vi "Test_pgADONet.vi"() -> ()   [LabVIEW 2026]
uses:
  <vilib>/Viviota/shared/ORM.lvlibp/TypeMap/TypeMap.lvclass
  <vilib>/Viviota/shared/ORM_ADONetCore.lvlibp/ADOMapper/ADOMapper.lvclass
  C:/Program Files/National Instruments/LabVIEW 2026/vi.lib/Viviota/shared/ORM.lvlibp/SqlMapper/SqlMapper.lvclass
  dotNetCore/ORM_DBC_Npgsql_netCore/DBC.lvclass
  C:/Program Files/National Instruments/LabVIEW 2026/vi.lib/Viviota/shared/ORM.lvlibp/DbConnection/DbConnection.lvclass
  <vilib>/Viviota/shared/ORM_lib.lvlibp/ObjectRow/ObjectLUT.lvclass
  <vilib>/numeric/Random Number (Range) I64.vi
  <vilib>/numeric/Random Number (Range) DBL.vi
  f3693442-7653-4e44-a421-498bef5f0c13.vi
  <vilib>/Analysis/baseanly.llb/Mean (DBL).vi
  <vilib>/numeric/sub_Random U32.vi
  <vilib>/JDP Science/JSONtext/Variant to JSON Text.vi
  <vilib>/Viviota/shared/ORM_lib.lvlibp/ObjectRow/Write LUT.vi
  <vilib>/Viviota/shared/ORM.lvlibp/DbConnection/Write SupportTX.vi
  <vilib>/Viviota/shared/ORM.lvlibp/SqlMapper/Write DbConnection.vi
  <vilib>/Viviota/shared/ORM.lvlibp/TypeMap/Write Table Name.vi
  <vilib>/Viviota/shared/ORM.lvlibp/TypeMap/Write Autokey.vi
  <vilib>/Viviota/shared/ORM_lib.lvlibp/ObjectRow/Read LUT.vi
  <vilib>/JDP Science/JSONtext/LVClass Serializer/JSONtext LVClass Serializer.lvclass
  <vilib>/Analysis/NI_AALBase.lvlib
panel:
  out "Numeric 2":i32
  out "Numeric":i32
  out "mean 3":dbl format="%0.6f"
  out "mean 2":dbl format="%0.6f"
  out "mean":dbl format="%0.6f"
  out "x-y":dbl[](array[numeric])
  out "Array 2":dbl[](array[numeric])
  out "Array":dbl[](array[numeric])
  out "LUT 2":variant[](array[variant])
  out "LUT":variant[](array[variant])
  out "id":i32[](array[numeric])
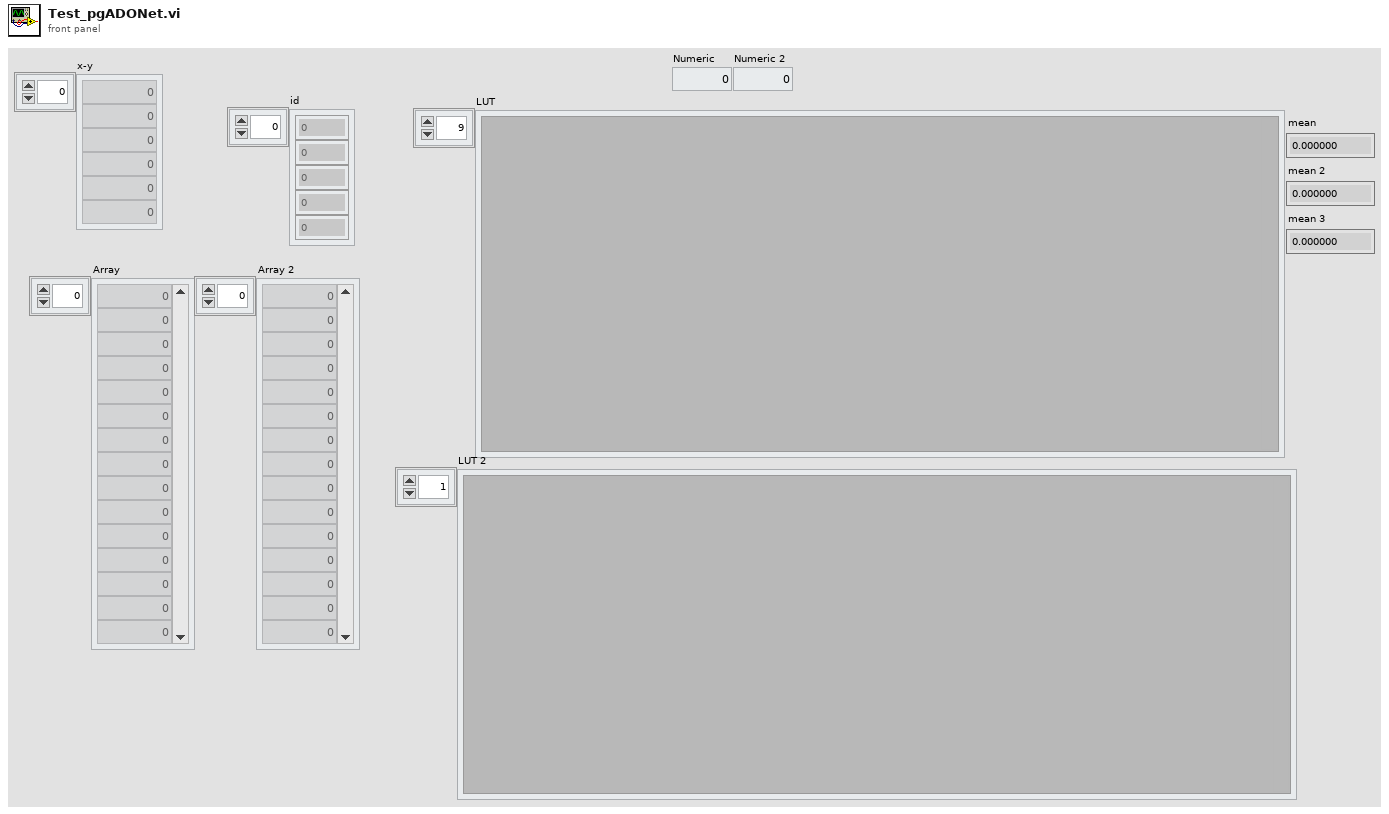
[diagram p1: front panel]
types:
  T1 = cluster{"Text":string, "Integer":i32, "dbl":dbl, "timestamp":timestamp}
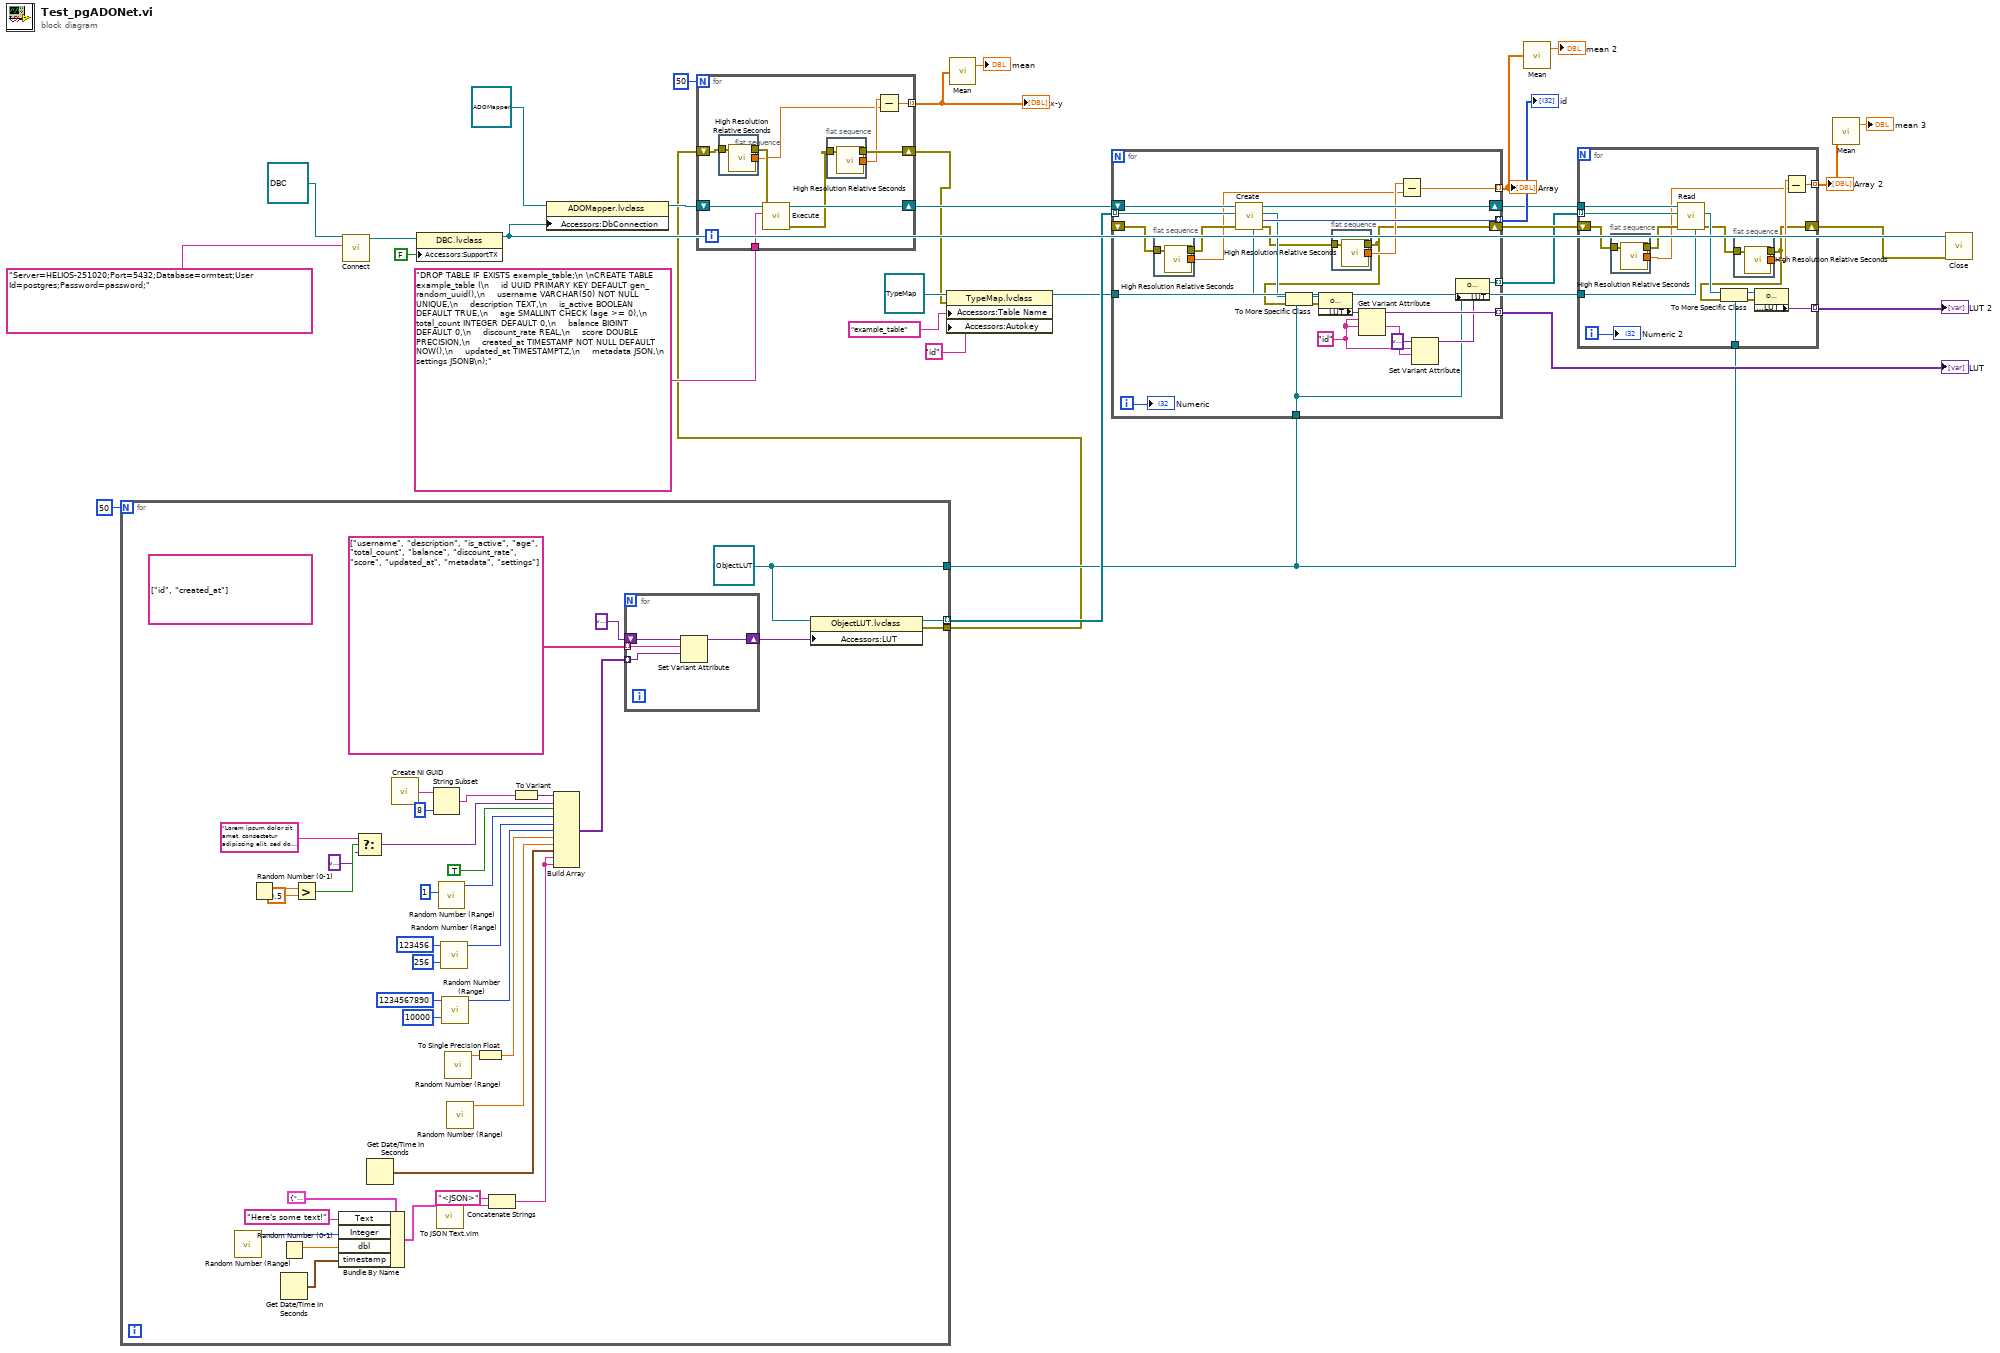
[diagram p0: block diagram]
diagram:
  n1 = for {
    N: 50 -> [_]
    tunnel: [w39] -> w26 mode=indexing
    tunnel: [w38] -> w16
    tunnel: [w33] -> w11
    w38 = refnum<class "ObjectLUT.lvclass"> refnum ("ORM_lib.lvlibp:ObjectLUT.lvclass")
    (unwired) string[] ["id", "created_at"]
    n2 = call-poly <vilib>:"Random Number (Range).vi"() -> ("number"=w46:i64)  [unwired: 11 in]
    n3 = Random Number (0-1)() -> (number: 0 to 1=w55:dbl)
    n4 = Random Number (0-1)() -> (number: 0 to 1=w47:dbl)
    n5 = Get Date/Time In Seconds() -> (seconds since 1Jan1904=w48:timestamp)
    n6 = Greater?(x=w55, y=0.5) -> (0:w53:bool)
    n7 = Bundle By Name(cluster=T1 {"Text"="This is a test", "Integer"=0, "dbl"=0.0, "timestamp"=timestamp(0 s since 1904-01-01)}, "Text"="Here's some text!", "Integer"=w46, "dbl"=w47, "timestamp"=w48) -> (w44:T1)
    n8 = Select(t="Lorem ipsum dolor sit amet, consectetur adipiscing elit, sed do eiusmod tempor incididunt ut labore et dolore magna aliqua", s=w53, f=variant) -> (s? t:f=w51:variant)
    n9 = Get Date/Time In Seconds() -> (seconds since 1Jan1904=w45:timestamp)
    n10 = call <vilib>:"Create NI GUID.vi"() -> ("NI GUID"=w71:string)
    n11 = String Subset(string=w71, length (rest)=8 ("length (rest)")) -> (substring=w66:string)  [unwired: 1 in]
    n12 = call "To JSON Text.vim"("Anything"=w44) -> ("<JSON>"=w37:string)  [unwired: 9 in, 1 out]
    n13 = call-poly <vilib>:"Random Number (Range).vi"("lower bound (-100)"=i64 1) -> ("number"=w63:i64)  [unwired: 10 in]
    n14 = call-poly <vilib>:"Random Number (Range).vi"("lower bound (-100)"=i64 256, "upper bound (100)"=i64 123456) -> ("number"=w62:i64)  [unwired: 9 in]
    n15 = call-poly <vilib>:"Random Number (Range).vi"("lower bound (-100)"=i64 10000, "upper bound (100)"=i64 1234567890) -> ("number"=w61:i64)  [unwired: 9 in]
    n16 = call-poly <vilib>:"Random Number (Range).vi"() -> ("number"=w59:dbl)  [unwired: 11 in]
    n17 = call-poly <vilib>:"Random Number (Range).vi"() -> ("number"=w57:dbl)  [unwired: 11 in]
    n18 = To Single Precision Float(number=w59) -> (single precision float=w58:sgl)
    n19 = Concatenate Strings("<JSON>" ("string"), w37) -> (w36:string)
    n20 = To Variant(anything=w66) -> (Variant=w65:variant)
    n21 = Build Array(w65, w51, TRUE, w63, w62, w61, w58, w57, w45, w36, w36) -> (w42:variant[])
    n22 = for {
      tunnel: string[] ["username", "description", "is_active", "age", "total_count", "balance", "discount_rate", "score", "updated_at", "metadata", "settings"] -> [w75] mode=indexing
      tunnel: w42 -> [w74] mode=indexing
      shift-right: [w73] -> w40
      shift-left: variant -> [w72]
      n23 = Set Variant Attribute(Variant=w72, name=w75, value=w74) -> (Variant out=w73:variant)  [unwired: 1 in, 2 out]
    }
    n24 = property class="ObjectLUT.lvclass"(reference=w38, "Accessors:LUT"=w40) -> (reference out=w39:refnum<class "ObjectLUT.lvclass">, error out=w33:errorcluster)  [unwired: 1 in]
  }
  n25 = call-dynamic "Connect.vi"("Connection String"="Server=HELIOS-251020;Port=5432;Database=ormtest;User Id=postgres;Password=password;", "PostgresqlConnection in"=refnum<class "DBC.lvclass"> refnum ("ORM_DBC_Npgsql_netCore.lvlib:DBC.lvclass")) -> ("PostgresqlConnection out"=w31:refnum<class "DBC.lvclass">)  [unwired: 8 in, 1 out]
  n26 = property class="DBC.lvclass"(reference=w31, "Accessors:SupportTX"=FALSE ("SupportTX")) -> (reference out=w27:refnum<class "DBC.lvclass">)  [unwired: 1 in, 1 out]
  n27 = property class="ADOMapper.lvclass"(reference=refnum<class "ADOMapper.lvclass"> refnum ("ORM_ADONetCore.lvlibp:ADOMapper.lvclass"), "Accessors:DbConnection"=w27) -> (reference out=w29:refnum<class "ADOMapper.lvclass">)  [unwired: 1 in, 1 out]
  n28 = for {
    N: 50 -> [_]
    tunnel: "DROP TABLE IF EXISTS example_table;\n \nCREATE TABLE example_table (\n    id UUID PRIMARY KEY DEFAULT gen_random_uuid(),\n    username VARCHAR(50) NOT NULL UNIQUE,\n    description TEXT,\n    is_active BOOLEAN DEFAULT TRUE,\n    age SMALLINT CHECK (age >= 0),\n    total_count INTEGER DEFAULT 0,\n    balance BIGINT DEFAULT 0,\n    discount_rate REAL,\n    score DOUBLE PRECISION,\n    created_at TIMESTAMP NOT NULL DEFAULT NOW(),\n    updated_at TIMESTAMPTZ,\n    metadata JSON,\n    settings JSONB\n);" ("sql") -> [w84]
    tunnel: [w76] -> w7 mode=indexing
    shift-right: [w83] -> w18
    shift-left: w29 -> [w85]
    shift-right: [w79] -> w10
    shift-left: w11 -> [w82]
    n29 = flat-sequence {
      tunnel: [w89] -> w77
      tunnel: w82 -> [w88]
      tunnel: [w88] -> w81
      frame #0 {
        n30 = call <vilib>:"High Resolution Relative Seconds.vi"() -> ("relative seconds"=w89:dbl)
      }
    }
    n31 = call-dynamic "Execute.vi"("error in (no error)"=w81, "sql"=w84, "ADOMapper in"=w85) -> ("error out"=w80:errorcluster, "ADOMapper out"=w83:refnum<class "ADOMapper.lvclass">)  [unwired: 6 in, 1 out]
    n32 = flat-sequence {
      tunnel: [w87] -> w78
      tunnel: w80 -> [w86]
      tunnel: [w86] -> w79
      frame #0 {
        n33 = call <vilib>:"High Resolution Relative Seconds.vi"() -> ("relative seconds"=w87:dbl)
      }
    }
    n34 = Subtract(x=w78, y=w77) -> (x-y=w76:dbl)
  }
  "x-y" <- w7
  n35 = property class="TypeMap.lvclass"(reference=refnum<class "TypeMap.lvclass"> refnum ("TypeMap in"), error in=w10, "Accessors:Table Name"="example_table" ("Table Name"), "Accessors:Autokey"="id" ("Autokey")) -> (reference out=w17:refnum<class "TypeMap.lvclass">)  [unwired: 1 out]
  n36 = call-poly <vilib>:"Mean.vi"("X"=w7) -> ("mean"=→"mean":dbl)  [unwired: 1 out]
  n37 = for {
    tunnel: w26 -> [w112] mode=indexing
    tunnel: w17 -> [w111]
    tunnel: [w110] -> w23 mode=indexing
    tunnel: w16 -> [w100]
    tunnel: [w105] -> w22 mode=indexing
    shift-right: [w91] -> w20
    shift-left: _ -> [w98]
    tunnel: [w99] -> w19 mode=indexing
    shift-right: [w95] -> w12
    shift-left: w18 -> [w113]
    tunnel: [w92] -> w4 mode=indexing
    i -> [w90]
    w103 = "id" ("name")
    n38 = flat-sequence {
      tunnel: [w117] -> w93
      tunnel: w98 -> [w116]
      tunnel: [w116] -> w97
      frame #0 {
        n39 = call <vilib>:"High Resolution Relative Seconds.vi"() -> ("relative seconds"=w117:dbl)
      }
    }
    n40 = call-dynamic "Create.vi"("TypeMap in"=w111, "error in (no error)"=w97, "object in"=w112, "SqlMapper in"=w113) -> ("error out"=w96:errorcluster, "id"=w110:i32, "object out"=w109:refnum<class>, "SqlMapper out"=w95:refnum<class "SqlMapper.lvclass">)  [unwired: 4 in]
    n41 = To More Specific Class(target class=w100, reference=w109, error in=w91) -> (specific class reference=w107:refnum<class "ObjectLUT.lvclass">, error out=w108:errorcluster)
    n42 = property class="ObjectLUT.lvclass"(reference=w107, error in=w108) -> ("Accessors:LUT"=w106:variant)  [unwired: 2 out]
    n43 = flat-sequence {
      tunnel: [w115] -> w94
      tunnel: w96 -> [w114]
      tunnel: [w114] -> w91
      frame #0 {
        n44 = call <vilib>:"High Resolution Relative Seconds.vi"() -> ("relative seconds"=w115:dbl)
      }
    }
    n45 = Get Variant Attribute(Variant=w106, name=w103, default value (empty Variant)=w103) -> (duplicate Variant=w105:variant, value=w102:string)  [unwired: 1 in, 2 out]
    n46 = Subtract(x=w94, y=w93) -> (x-y=w92:dbl)
    n47 = Set Variant Attribute(Variant=variant ("variant"), name=w103, value=w102) -> (Variant out=w101:variant)  [unwired: 1 in, 2 out]
    n48 = property class="ObjectLUT.lvclass"(reference=w100, "Accessors:LUT"=w101) -> (reference out=w99:refnum<class "ObjectLUT.lvclass">)  [unwired: 1 in, 1 out]
    "Numeric" <- w90
  }
  "id" <- w23
  "LUT" <- w22
  "Array" <- w4
  n49 = call-poly <vilib>:"Mean.vi"("X"=w4) -> ("mean"=→"mean 2":dbl)  [unwired: 1 out]
  n50 = for {
    tunnel: w19 -> [w133] mode=indexing
    tunnel: w12 -> [w132]
    tunnel: w17 -> [w131]
    tunnel: w16 -> [w127]
    tunnel: [w126] -> w15 mode=indexing
    shift-right: [w119] -> w14
    shift-left: w20 -> [w125]
    tunnel: [w120] -> w3 mode=indexing
    i -> [w118]
    n51 = flat-sequence {
      tunnel: [w137] -> w121
      tunnel: w125 -> [w136]
      tunnel: [w136] -> w124
      frame #0 {
        n52 = call <vilib>:"High Resolution Relative Seconds.vi"() -> ("relative seconds"=w137:dbl)
      }
    }
    n53 = call-dynamic "Read.vi"("TypeMap in"=w131, "error in (no error)"=w124, "object in"=w133, "SqlMapper in"=w132) -> ("error out"=w123:errorcluster, "Value"=w128:refnum<class>)  [unwired: 4 in, 2 out]
    n54 = To More Specific Class(target class=w127, reference=w128, error in=w119) -> (specific class reference=w130:refnum<class "ObjectLUT.lvclass">, error out=w129:errorcluster)
    n55 = flat-sequence {
      tunnel: [w135] -> w122
      tunnel: w123 -> [w134]
      tunnel: [w134] -> w119
      frame #0 {
        n56 = call <vilib>:"High Resolution Relative Seconds.vi"() -> ("relative seconds"=w135:dbl)
      }
    }
    n57 = property class="ObjectLUT.lvclass"(reference=w130, error in=w129) -> ("Accessors:LUT"=w126:variant)  [unwired: 2 out]
    n58 = Subtract(x=w122, y=w121) -> (x-y=w120:dbl)
    "Numeric 2" <- w118
  }
  "LUT 2" <- w15
  "Array 2" <- w3
  n59 = call-poly <vilib>:"Mean.vi"("X"=w3) -> ("mean"=→"mean 3":dbl)  [unwired: 1 out]
  n60 = call-dynamic "Close.vi"("error in (no error)"=w14, "dbcDotNet in"=w27) -> ()  [unwired: 9 in, 1 out]
